vi "test bin file.vi"() -> ()   [LabVIEW 2013, in "Binary logger tests.lvlib"]
uses:
  Binary logger tests.lvlib
  <vilib>/NI/Tag Bus/tag/Data Type.ctl
  <vilib>/NI/Tag Bus Module Framework/channel/channel classification.ctl
  <vilib>/NI/Tag Bus/tag/tag descriptor.lvclass/tag descriptor.ctl
  <vilib>/NI/Tag Bus/dictionary/data dictionary.lvclass/data dictionary.ctl
  execution/data cache.ctl
  <vilib>/NI/Tag Bus/table/data table.ctl
  <vilib>/NI/Tag Bus/tag/write raw default value.vi
  <vilib>/NI/Configuration Framework/serializable configuration/NISE_CEF_serializable configuration.lvclass
  execution/Binary datalogger runtime.lvclass
  <vilib>/NI/Tag Bus/dictionary/data dictionary.lvclass
  <vilib>/NI/Tag Bus/table/data table.lvlib
  <vilib>/NI/Tag Bus Module Framework/channel/TBM channel.lvclass
  <vilib>/NI/Tag Bus/tag/tag descriptor.lvclass
panel:
  out "empty?":bool
  out "x = y? 3":bool
  out "x = y? 2":bool
  out "x = y?":bool
  out "del error":errorcluster
  out "error out":errorcluster
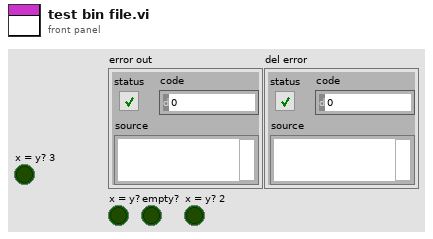
[diagram p1: front panel]
types:
  T1 = typedef "tag bus.lvlib/tag descriptor.lvclass/Data Type.ctl" = enum16{"Double", "Single", "I64", "I32", "I16", "I8", "U64", "U32", "U16", "U8", "Boolean", "String", "Array of Double", "Array of Single", "Array of I64", "Array of I32", "Array of I16", "Array of I8", "Array of U64", "Array of U32", "Array of U16", "Array of U8", "Array of Boolean", "Array of String"}
  T2 = typedef "TBM channel.lvclass/channel classification.ctl" = enum16{"input data", "output data", "processing parameter", "processing result"}
  T3 = enum16{"open", "replace", "create", "open or create", "replace or create", "replace or create with confirmation"}
  T4 = typedef "tag bus.lvlib/data dictionary.lvclass/full data dictionary.ctl" = cluster{"Double":string[], "Single":string[], "I64":string[], "I32":string[], "I16":string[], "I8":string[], "U64":string[], "U32":string[], "U16":string[], "U8":string[], "Boolean":string[], "String":string[], "Array of Double":string[], "Array of Single":string[], "Array of I64":string[], "Array of I32":string[], "Array of I16":string[], "Array of I8":string[], "Array of U64":string[], "Array of U32":string[], "Array of U16":string[], "Array of U8":string[], "Array of Boolean":string[], "Array of String":string[]}
  T5 = typedef "tag bus.lvlib/data table.lvlib/data table.ctl" = cluster{"Double":dbl[], "Single":sgl[], "I64":i64[], "I32":i32[], "I16":i16[], "I8":i8[], "U64":u64[], "U32":u32[], "U16":u16[], "U8":u8[], "Boolean":bool[], "String":string[], "Array of Double":cluster{"DBL Array":dbl[]}[], "Array of Single":cluster{"SGL Array":sgl[]}[], "Array of I64":cluster{"I64 Array":i64[]}[], "Array of I32":cluster{"I32 Array":i32[]}[], "Array of I16":cluster{"I16 Array":i16[]}[], "Array of I8":cluster{"I8 Array":i8[]}[], "Array of U64":cluster{"U64 Array":u64[]}[], "Array of U32":cluster{"U32 Array":u32[]}[], "Array of U16":cluster{"U16 Array":u16[]}[], "Array of U8":cluster{"U8 Array":u8[]}[], "Array of Boolean":cluster{"Boolean Array":bool[]}[], "Array of String":cluster{"String Array":string[]}[]}
  T6 = typedef "Binary datalogger runtime.lvclass/data cache.ctl" = cluster{"timestamps":timestamp[], "dataset":T5[]}
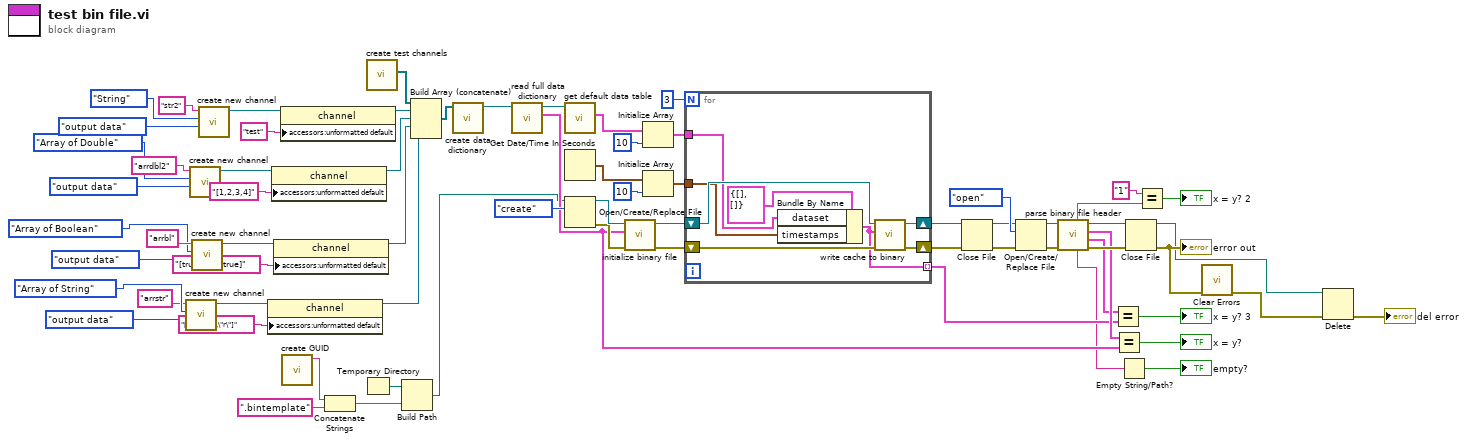
[diagram p0: block diagram]
diagram:
  n1 = call <vilib>:"create new channel.vi"("channel classification"=channel_classification."output data", "data type"=Data_Type."Array of String", "channel name"="arrstr") -> ("channel"=w3:refnum<class "TBM channel.lvclass">)  [unwired: 8 in]
  n2 = call <vilib>:"create new channel.vi"("channel classification"=channel_classification."output data", "data type"=Data_Type."Array of Double", "channel name"="arrdbl2") -> ("channel"=w15:refnum<class "TBM channel.lvclass">)  [unwired: 8 in]
  n3 = call <vilib>:"create new channel.vi"("channel classification"=channel_classification."output data", "data type"=Data_Type."Array of Boolean", "channel name"="arrbl") -> ("channel"=w13:refnum<class "TBM channel.lvclass">)  [unwired: 8 in]
  n4 = call <vilib>:"create new channel.vi"("channel classification"=channel_classification."output data", "data type"=Data_Type."String", "channel name"="str2") -> ("channel"=w25:refnum<class "TBM channel.lvclass">)  [unwired: 8 in]
  n5 = property class="channel"(reference=w3, "accessors:unformatted default"="[\"s\",\"t\",\"r\"]" ("unformatted default")) -> (reference out=w2:refnum<class "TBM channel.lvclass">)  [unwired: 1 in, 1 out]
  n6 = property class="channel"(reference=w15, "accessors:unformatted default"="[1,2,3,4]" ("unformatted default")) -> (reference out=w14:refnum<class "TBM channel.lvclass">)  [unwired: 1 in, 1 out]
  n7 = property class="channel"(reference=w13, "accessors:unformatted default"="[true,false,true]" ("unformatted default")) -> (reference out=w10:refnum<class "TBM channel.lvclass">)  [unwired: 1 in, 1 out]
  n8 = property class="channel"(reference=w25, "accessors:unformatted default"="test" ("unformatted default")) -> (reference out=w21:refnum<class "TBM channel.lvclass">)  [unwired: 1 in, 1 out]
  n9 = call <vilib>:"create GUID.vi"() -> ("uuid"=w68:string)  [unwired: 10 in, 1 out]
  n10 = Concatenate Strings(w68, ".bintemplate" ("string")) -> (w66:string)
  n11 = Temporary Directory() -> (w69:path)
  n12 = call "create test channels.vi"() -> ("chans"=w42:refnum<class "TBM channel.lvclass">[])  [unwired: 8 in, 3 out]
  n13 = Build Path(base path=w69, name or relative path=w66) -> (appended path=w1:path)
  n14 = Build Array (concatenate)(w42, w21, w14, w10, w2) -> (w26:refnum<class "TBM channel.lvclass">[])
  n15 = call <vilib>:"create data dictionary.vi"("system tags"=w26) -> ("data dictionary"=w41:refnum<class "data dictionary.lvclass">)  [unwired: 9 in, 1 out]
  n16 = call <vilib>:"read full data dictionary.vi"("data dictionary in"=w41) -> ("dictionary"=w40:T4, "data dictionary out"=w39:refnum<class "data dictionary.lvclass">)  [unwired: 8 in, 1 out]
  n17 = call <vilib>:"get default data table.vi"("data dictionary in"=w39) -> ("default data table"=w38:T5)  [unwired: 9 in, 1 out]
  n18 = Get Date/Time In Seconds() -> (seconds since 1Jan1904=w35:timestamp)
  n19 = Open/Create/Replace File(file path (use dialog)=w1, operation (0:open)=T3."create") -> (refnum out=w64:refnum<file>, error out=w63:errorcluster)  [unwired: 4 in, 1 out]
  n20 = call "initialize binary file.vi"("error in"=w63, "dictionary"=w40, "Byte Stream File in"=w64) -> ("error out"=w43:errorcluster, "Byte Stream File out"=w46:refnum<file>)  [unwired: 7 in]
  n21 = Initialize Array(w38, 10 ("dimension size")) -> (w34:T5[])
  n22 = Initialize Array(w35, 10 ("dimension size")) -> (w33:timestamp[])
  n23 = for {
    N: 3 -> [_]
    shift-right: [w76] -> w45
    shift-left: w46 -> [w77]
    shift-right: [w75] -> w44
    shift-left: w43 -> [w74]
    tunnel: w34 -> [w72]
    tunnel: w33 -> [w71]
    tunnel: [w70] -> w30 mode=indexing
    n24 = Bundle By Name(cluster=T6 {"timestamps"=[], "dataset"=[]} ("cache in"), "dataset"=w72, "timestamps"=w71) -> (w70:T6)
    n25 = call "write cache to binary.vi"("error in"=w74, "cache in"=w70, "bin file in"=w77) -> ("error out"=w75:errorcluster, "bin file out"=w76:refnum<file>)  [unwired: 6 in, 1 out]
  }
  n26 = Close File(refnum=w45, error in=w44) -> (path=w61:path, error out=w60:errorcluster)
  n27 = Open/Create/Replace File(file path (use dialog)=w61, error in=w60, operation (0:open)=T3."open") -> (refnum out=w55:refnum<file>, error out=w52:errorcluster)  [unwired: 3 in, 1 out]
  n28 = call "parse binary file header.vi"("error in"=w52, "Byte Stream File in"=w55) -> ("error out"=w53:errorcluster, "data"=w29:T6[], "dictionary"=w51:T4, "Byte Stream File out"=w54:refnum<file>, "remaining string"=w28:string, "version"=w49:string)  [unwired: 4 in]
  n29 = Equal?(x=w29, y=w30) -> (x = y?=→"x = y? 3":bool)
  n30 = Equal?(x=w51, y=w40) -> (x = y?=→"x = y?":bool)
  n31 = Empty String/Path?(string/path=w28) -> (empty?=→"empty?":bool)
  n32 = Close File(refnum=w54, error in=w53) -> (path=w58:path, error out=w59:errorcluster)
  "error out" <- w59
  n33 = Equal?(x="1", y=w49) -> (x = y?=→"x = y? 2":bool)
  n34 = call <vilib>:"Clear Errors.vi"("error in (no error)"=w59) -> ("error out"=w57:errorcluster)  [unwired: 6 in]
  n35 = Delete(path (use dialog)=w58, error in=w57) -> (error out=→"del error":errorcluster)  [unwired: 3 in, 2 out]
